vi "Set Query (attributes).vi"(8 "error in (no error)":errorcluster, 10 "Query":variant, 11 "URI in":refnum<class "URI.lvclass">) -> (0 "error out":errorcluster, 3 "URI out":refnum<class "URI.lvclass">)   [LabVIEW 2013, in "openURI.lvlib" / "URI.lvclass"]
doc: "The Query variant input must contain attributes of type \"string\".\nAll data contained in the variant will be ignored. All attributes that are not of type \"string\" will be ignored."
uses:
  URI.lvclass
  URI.lvclass/URI.ctl
  components/query/URI-Component.Query.lvclass
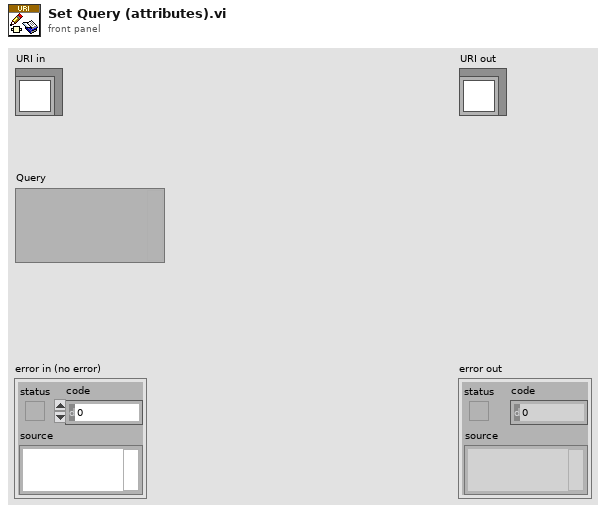
[diagram p1: front panel]
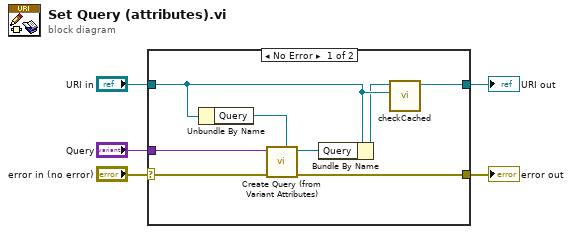
[diagram p0: block diagram]
diagram:
  n1 = case shown="No Error" "error in (no error)" {
    selector: "error in (no error)" -> [w12 w15]
    tunnel: [w11 w15] -> w4
    tunnel: [w6 w14] -> w2
    tunnel: "URI in" -> [w8 w14]
    tunnel: "Query" -> [w13 _]
    frame No Error {
      n2 = Unbundle By Name(w8) -> ("Query"=w9:refnum<class "URI-Component.Query.lvclass">)
      n3 = call "Create Query (from Variant Attributes).vi"("URI-Component.Query"=w9, "error in (no error)"=w12, "Query"=w13) -> ("error out"=w11:errorcluster, "URI-Component.Query"=w10:refnum<class "URI-Component.Query.lvclass">)  [unwired: 7 in]
      n4 = Bundle By Name(cluster=w8, "Query"=w10) -> (w7:refnum<class "URI.lvclass">)
      n5 = call "checkCached.vi"("Old"=w8, "New URI"=w7) -> ("URI"=w6:refnum<class "URI.lvclass">)  [unwired: 9 in]
    }
    frame Error {
    }
  }
  "error out" <- w4
  "URI out" <- w2
